vi "Measurement Logic.vi"() -> ()   [LabVIEW 2021, in "PSRR_PMIC.lvlib"]
uses:
  PSRR_PMIC.lvlib
  <vilib>/Plug-In SDKs/Measurements/Measure Call Context/Measure Call Context.lvclass
  Measurement Configuration.ctl
  Measurement Results.ctl
  <instrlib>/niDCPower/nidcpower.llb/niDCPower Output Function.ctl
  <instrlib>/niDCPower/nidcpower.llb/niDCPower Wait For Event - Event.ctl
  <instrlib>/niDCPower/nidcpower.llb/niDCPower Source Mode.ctl
  <instrlib>/niFgen/niFgen.llb/niFgen Output Mode.ctl
  <instrlib>/niScope/Controls/niScope vertical coupling.ctl
  <instrlib>/niScope/Controls/niScope trigger slope.ctl
  <instrlib>/niScope/Controls/niScope trigger coupling.ctl
  <instrlib>/niScope/Controls/niScope trigger source.ctl
  <instrlib>/niDCPower/nidcpower.llb/niDCPower Get Channel Name From String.vi
  <instrlib>/niScope/Utility/niScope Get Channel Name From String.vi
  <instrlib>/niScope/Configure/Trigger/niScope Configure Trigger Edge.vi
panel:
  out "measurement results":T1
  in  "measurement configuration":T2={"DUT setup time"=1.0, "Source resource name"="", "Source sense"=1009, "Source current limit"=0.15, "Source voltage level"=10.0, "Load resource name"="", "Load sense"=1009, "Load voltage limit range"=6.0, "Load current level"=0.025, "Fgen resource name"="", "Fgen channel name"="", "Fgen pk-pk amplitude"=1.0, "Fgen load impedance"=10000.0, "Fgen start frequency"=10.0, "Fgen stop frequency"=10000000.0, "Fgen frequency sweep points/points per decade"=10, "Fgen sweep type"="Logarithmic", "Fgen standard Waveform"=enum."Sine", "Scope resource name"="", "Scope input channel name"="", "Scope output channel name"="", "Scope probe attenuation"=1.0, "Scope samples per cycle"=1000, "Scope cycles to average"=4} {"Fgen stop frequency" format="%#_6p"; "Fgen pk-pk amplitude" format="%#_6p"; "Load sense" items=["Local"=1008, "Remote"=1009]; "Source sense" items=["Local"=1008, "Remote"=1009]}
  out "measure call context out":refnum<class "Measure Call Context.lvclass">
  in  "measure call context in":refnum<class "Measure Call Context.lvclass">
  out "error out":errorcluster
  in  "error in":errorcluster
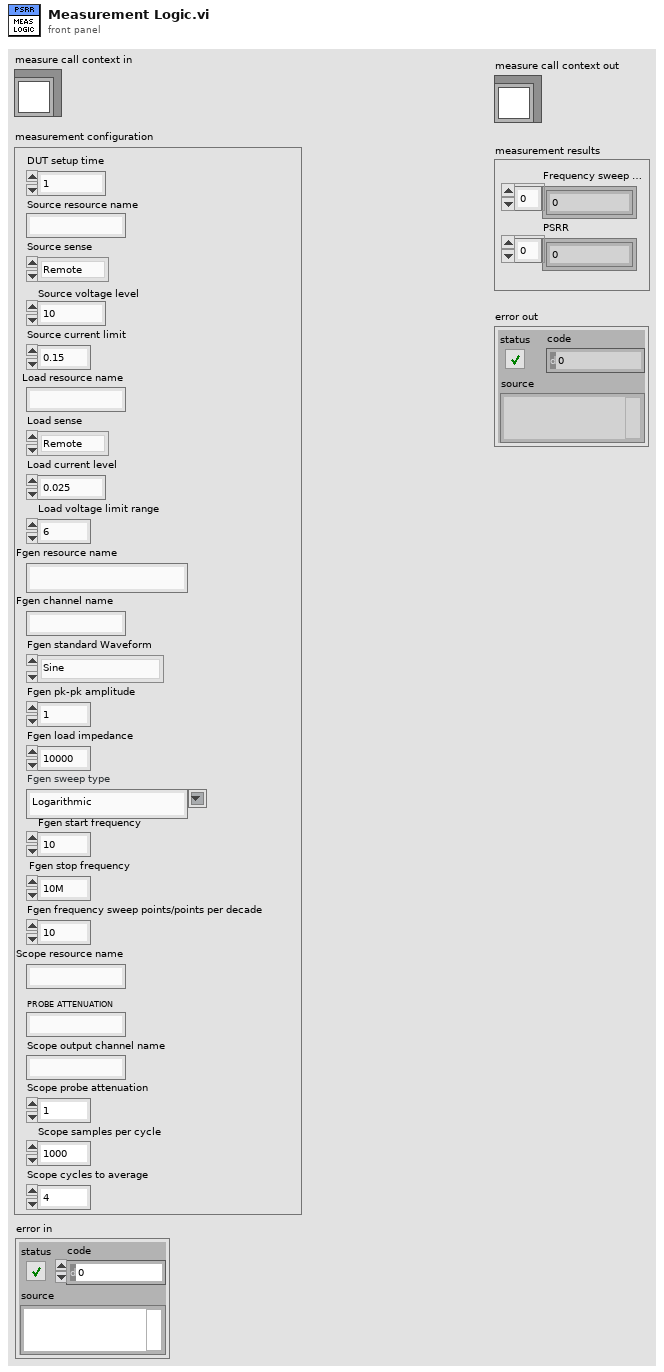
[diagram p1: front panel]
types:
  T1 = typedef "PSRR_PMIC.lvlib/Measurement Results.ctl" = cluster{"Frequency sweep points":dbl[], "PSRR":dbl[]}
  T2 = typedef "PSRR_PMIC.lvlib/Measurement Configuration.ctl" = cluster{"DUT setup time":dbl, "Source resource name":string, "Source sense":i32, "Source current limit":dbl, "Source voltage level":dbl, "Load resource name":string, "Load sense":i32, "Load voltage limit range":dbl, "Load current level":dbl, "Fgen resource name":string, "Fgen channel name":string, "Fgen pk-pk amplitude":dbl, "Fgen load impedance":dbl, "Fgen start frequency":dbl, "Fgen stop frequency":dbl, "Fgen frequency sweep points/points per decade":i32, "Fgen sweep type":string, "Fgen standard Waveform":enum32{"Sine", "Square", "Triangle", "Ramp Up", "Ramp Down", "DC", "Noise"}, "Scope resource name":string, "Scope input channel name":string, "Scope output channel name":string, "Scope probe attenuation":dbl, "Scope samples per cycle":i32, "Scope cycles to average":i32}
  T3 = typedef "niScope trigger coupling.ctl" = u16
  T4 = typedef "niScope trigger slope.ctl" = i32
  T5 = typedef "niScope vertical coupling.ctl" = i32
  T6 = typedef "niFgen Output Mode.ctl" = u32
  T7 = typedef "niDCPower Output Function.ctl" = i32
  T8 = typedef "niDCPower Source Mode.ctl" = i32
  T9 = typedef "niDCPower Wait For Event - Event.ctl" = i32
  T10 = enum32{"Sine", "Square", "Triangle", "Ramp Up", "Ramp Down", "DC", "Noise"}
  T11 = typedef "niScope trigger source.ctl" = string
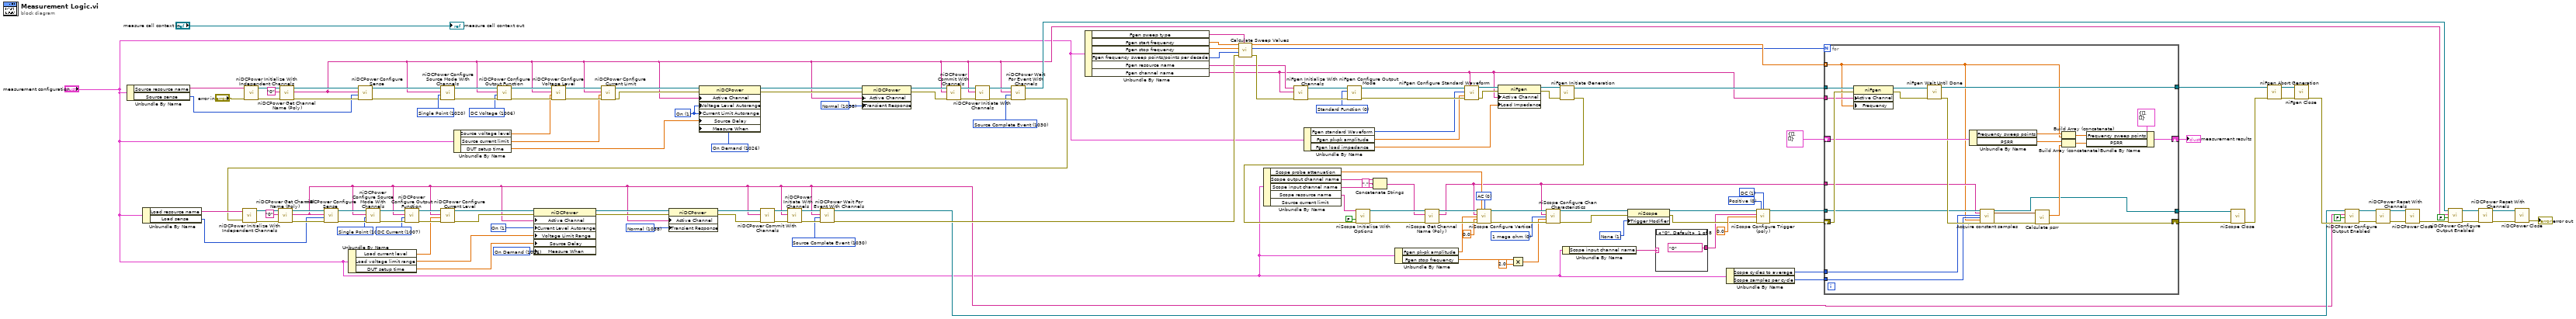
[diagram p0: block diagram]
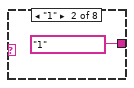
[diagram p2: hidden frame]
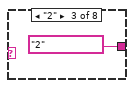
[diagram p3: hidden frame]
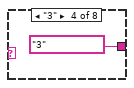
[diagram p4: hidden frame]
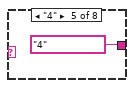
[diagram p5: hidden frame]
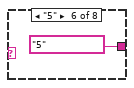
[diagram p6: hidden frame]
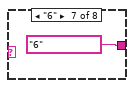
[diagram p7: hidden frame]
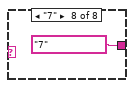
[diagram p8: hidden frame]
diagram:
  w53 = 1 items=["None"=1, "Auto Trigger"=2] ("Triggering:Trigger Modifier")
  w59 = T3 1 items=["AC"=0, "DC"=1, "HF Reject"=3, "LF Reject"=4, "AC Plus HF Reject"=1001] ("trigger coupling")
  w60 = T4 0 items=["Positive", "Negative"] ("trigger slope")
  w62 = T5 0 items=["AC", "DC", "Ground"] ("vertical coupling")
  w65 = u32 0 items=["1 mega ohm"=0, "50 ohms"=2] ("input impedance")
  w81 = T6 0 items=["Standard Function", "Frequency List", "Arbitrary Waveform", "Arbitrary Sequence", "Script"] ("Output Mode (default: 0=Standard Function)")
  w100 = T7 1007 items=["DC Voltage"=1006, "DC Current"=1007, "Pulse Voltage"=1049, "Pulse Current"=1050] ("output function")
  w101 = T8 1020 items=["Single Point"=1020, "Sequence"=1021] ("source mode")
  w26 = 1026 items=["Automatically after Source Complete"=1025, "On Demand"=1026, "On Measure Trigger"=1027] ("Measurement:Advanced:Measure When")
  w103 = 1 items=["Off", "On"] ("Source:DC Current:Current Level Autorange")
  w115 = 1038 items=["Slow"=1041, "Normal"=1038, "Fast"=1039, "Custom"=1042] ("Source:Transient Response")
  w118 = T9 1030 items=["Source Complete Event"=1030, "Measure Complete Event"=1031, "Sequence Iteration Complete Event"=1032, "Sequence Engine Done Event"=1033, "Pulse Complete Event"=1051, "Ready For Pulse Trigger Event"=1052] ("event")
  w123 = T9 1030 items=["Source Complete Event"=1030, "Measure Complete Event"=1031, "Sequence Iteration Complete Event"=1032, "Sequence Engine Done Event"=1033, "Pulse Complete Event"=1051, "Ready For Pulse Trigger Event"=1052] ("event")
  w131 = 1038 items=["Slow"=1041, "Normal"=1038, "Fast"=1039, "Custom"=1042] ("Source:Transient Response")
  w138 = 1026 items=["Automatically after Source Complete"=1025, "On Demand"=1026, "On Measure Trigger"=1027] ("Measurement:Advanced:Measure When")
  w144 = 1 items=["Off", "On"] ("Source:DC Voltage:Current Limit Autorange")
  w146 = T7 1006 items=["DC Voltage"=1006, "DC Current"=1007, "Pulse Voltage"=1049, "Pulse Current"=1050] ("output function")
  w149 = T8 1020 items=["Single Point"=1020, "Sequence"=1021] ("source mode")
  n1 = Unbundle By Name("measurement configuration") -> ("Source resource name"=w150:string, "Source sense"=w1:i32)
  n2 = Unbundle By Name("measurement configuration") -> ("Load resource name"=w91:string, "Load sense"=w2:i32)
  n3 = call <instrlib>:"niDCPower Initialize With Independent Channels.vi"("error in (no error)"="error in", "resource name"=w150) -> ("error out"=w152:errorcluster, "instrument handle out"=w153:refnum<k15>)  [unwired: 8 in]
  n4 = call-poly <instrlib>:"niDCPower Get Channel Name (Poly).vi"("error in (no error)"=w152, "index"="0", "instrument handle"=w153) -> ("error out"=w121:errorcluster, "name"=w10:string, "instrument handle out"=w122:refnum<k15>)  [unwired: 6 in]
  n5 = Unbundle By Name("measurement configuration") -> ("Load current level"=w102:dbl, "Load voltage limit range"=w97:dbl, "DUT setup time"=w112:dbl)
  n6 = call <instrlib>:"niDCPower Configure Sense.vi"("error in (no error)"=w121, "sense"=w1, "channel name"=w10, "instrument handle"=w122) -> ("error out"=w130:errorcluster, "instrument handle out"=w129:refnum<k15>)  [unwired: 6 in]
  n7 = call <instrlib>:"niDCPower Configure Source Mode With Channels.vi"("error in (no error)"=w130, "source mode"=w149, "channel name"=w10, "instrument handle"=w129) -> ("error out"=w148:errorcluster, "instrument handle out"=w147:refnum<k15>)  [unwired: 6 in]
  n8 = Unbundle By Name("measurement configuration") -> ("Source voltage level"=w127:dbl, "Source current limit"=w128:dbl, "DUT setup time"=w126:dbl)
  n9 = call <instrlib>:"niDCPower Configure Output Function.vi"("error in (no error)"=w148, "output function"=w146, "channel name"=w10, "instrument handle"=w147) -> ("error out"=w142:errorcluster, "instrument handle out"=w141:refnum<k15>)  [unwired: 6 in]
  n10 = call <instrlib>:"niDCPower Configure Voltage Level.vi"("error in (no error)"=w142, "voltage level"=w127, "channel name"=w10, "instrument handle"=w141) -> ("error out"=w139:errorcluster, "instrument handle out"=w140:refnum<k15>)  [unwired: 6 in]
  n11 = call <instrlib>:"niDCPower Configure Current Limit.vi"("error in (no error)"=w139, "current limit"=w128, "channel name"=w10, "instrument handle"=w140) -> ("error out"=w145:errorcluster, "instrument handle out"=w143:refnum<k15>)  [unwired: 6 in]
  n12 = property class="niDCPower"(reference=w143, error in=w145, "Active Channel"=w10, "Voltage Level Autorange"=w144, "Current Limit Autorange"=w144, "Source Delay"=w126, "Measure When"=w138) -> (reference out=w135:refnum<k15>, error out=w134:errorcluster)
  n13 = property class="niDCPower"(reference=w135, error in=w134, "Active Channel"=w10, "Transient Response"=w131) -> (reference out=w133:refnum<k15>, error out=w132:errorcluster)
  n14 = call <instrlib>:"niDCPower Commit With Channels.vi"("error in (no error)"=w132, "channel name"=w10, "instrument handle"=w133) -> ("error out"=w136:errorcluster, "instrument handle out"=w137:refnum<k15>)  [unwired: 7 in]
  n15 = call <instrlib>:"niDCPower Initiate With Channels.vi"("error in (no error)"=w136, "channel name"=w10, "instrument handle"=w137) -> ("error out"=w124:errorcluster, "instrument handle out"=w125:refnum<k15>)  [unwired: 7 in]
  n16 = call <instrlib>:"niDCPower Wait For Event With Channels.vi"("error in (no error)"=w124, "event"=w123, "channel name"=w10, "instrument handle"=w125) -> ("error out"=w72:errorcluster, "instrument handle out"=w13:refnum<k15>)  [unwired: 6 in]
  n17 = call <instrlib>:"niDCPower Initialize With Independent Channels.vi"("error in (no error)"=w72, "resource name"=w91) -> ("error out"=w95:errorcluster, "instrument handle out"=w96:refnum<k15>)  [unwired: 8 in]
  n18 = call-poly <instrlib>:"niDCPower Get Channel Name (Poly).vi"("error in (no error)"=w95, "index"="0", "instrument handle"=w96) -> ("error out"=w92:errorcluster, "name"=w11:string, "instrument handle out"=w93:refnum<k15>)  [unwired: 6 in]
  n19 = call <instrlib>:"niDCPower Configure Sense.vi"("error in (no error)"=w92, "sense"=w2, "channel name"=w11, "instrument handle"=w93) -> ("error out"=w106:errorcluster, "instrument handle out"=w109:refnum<k15>)  [unwired: 6 in]
  n20 = call <instrlib>:"niDCPower Configure Source Mode With Channels.vi"("error in (no error)"=w106, "source mode"=w101, "channel name"=w11, "instrument handle"=w109) -> ("error out"=w105:errorcluster, "instrument handle out"=w108:refnum<k15>)  [unwired: 6 in]
  n21 = call <instrlib>:"niDCPower Configure Output Function.vi"("error in (no error)"=w105, "output function"=w100, "channel name"=w11, "instrument handle"=w108) -> ("error out"=w104:errorcluster, "instrument handle out"=w107:refnum<k15>)  [unwired: 6 in]
  n22 = call <instrlib>:"niDCPower Configure Current Level.vi"("error in (no error)"=w104, "current level"=w102, "channel name"=w11, "instrument handle"=w107) -> ("error out"=w98:errorcluster, "instrument handle out"=w99:refnum<k15>)  [unwired: 6 in]
  n23 = property class="niDCPower"(reference=w99, error in=w98, "Active Channel"=w11, "Current Level Autorange"=w103, "Voltage Limit Range"=w97, "Source Delay"=w112, "Measure When"=w26) -> (reference out=w114:refnum<k15>, error out=w113:errorcluster)
  n24 = property class="niDCPower"(reference=w114, error in=w113, "Active Channel"=w11, "Transient Response"=w115) -> (reference out=w111:refnum<k15>, error out=w110:errorcluster)
  n25 = call <instrlib>:"niDCPower Commit With Channels.vi"("error in (no error)"=w110, "channel name"=w11, "instrument handle"=w111) -> ("error out"=w116:errorcluster, "instrument handle out"=w117:refnum<k15>)  [unwired: 7 in]
  n26 = call <instrlib>:"niDCPower Initiate With Channels.vi"("error in (no error)"=w116, "channel name"=w11, "instrument handle"=w117) -> ("error out"=w120:errorcluster, "instrument handle out"=w119:refnum<k15>)  [unwired: 7 in]
  n27 = call <instrlib>:"niDCPower Wait For Event With Channels.vi"("error in (no error)"=w120, "event"=w118, "channel name"=w11, "instrument handle"=w119) -> ("error out"=w79:errorcluster, "instrument handle out"=w12:refnum<k15>)  [unwired: 6 in]
  n28 = Unbundle By Name("measurement configuration") -> ("Fgen sweep type"=w78:string, "Fgen start frequency"=w27:dbl, "Fgen stop frequency"=w77:dbl, "Fgen frequency sweep points/points per decade"=w76:i32, "Fgen resource name"=w8:string, "Fgen channel name"=w7:string)
  n29 = call "Calculate Sweep Values.vi"("Sweep type"=w78, "error in"=w79, "Points"=w76, "Stop level"=w77, "Start level"=w27) -> ("error out"=w80:errorcluster, "Sweep points"=w30:i32, "Sweep values"=w31:dbl[])  [unwired: 4 in]
  n30 = Unbundle By Name("measurement configuration") -> ("Scope probe attenuation"=w48:dbl, "Scope output channel name"=w45:string, "Scope input channel name"=w47:string, "Scope resource name"=w61:string)  [unwired: 1 out]
  n31 = call <instrlib>:"niFgen Initialize With Channels.vi"("error in (no error)"=w80, "Channel Name"=w7, "Resource Name"=w8) -> ("error out"=w86:errorcluster, "Instrument Handle Out"=w89:refnum<k15>)  [unwired: 7 in]
  n32 = Unbundle By Name("measurement configuration") -> ("Fgen standard Waveform"=w74:T10, "Fgen pk-pk amplitude"=w73:dbl, "Fgen load impedance"=w75:dbl)
  n33 = call <instrlib>:"niFgen Configure Output Mode.vi"("error in (no error)"=w86, "Output Mode (default: 0=Standard Function)"=w81, "Instrument Handle"=w89) -> ("error out"=w85:errorcluster, "Instrument Handle Out"=w88:refnum<k15>)  [unwired: 6 in]
  n34 = Concatenate Strings(w45, "," ("string"), w47) -> (w44:string)
  n35 = Unbundle By Name("measurement configuration") -> ("Fgen pk-pk amplitude"=w6:dbl, "Fgen stop frequency"=w51:dbl)
  n36 = call <instrlib>:"niFgen Configure Standard Waveform.vi"("Instrument Handle"=w88, "Channel Name"=w7, "Waveform"=w74, "Amplitude"=w73, "error in (no error)"=w85) -> ("Instrument Handle Out"=w87:refnum<k15>, "error out"=w84:errorcluster)  [unwired: 9 in]
  n37 = property class="niFgen"(reference=w87, error in=w84, "Active Channel"=w7, "Load Impedance"=w75) -> (reference out=w83:refnum<k15>, error out=w82:errorcluster)
  n38 = Multiply(x=w51, y=2.0) -> (x*y=w52:dbl)
  n39 = call <instrlib>:"niFgen Initiate Generation.vi"("error in (no error)"=w82, "Instrument Handle"=w83) -> ("error out"=w49:errorcluster, "Instrument Handle Out"=w32:refnum<k15>)  [unwired: 8 in]
  n40 = call <instrlib>:"niScope Initialize With Options.vi"("resource name"=w61, "reset device"=FALSE, "error in"=w49) -> ("instrument handle"=w71:refnum<k15>, "error out"=w68:errorcluster)  [unwired: 11 in]
  n41 = call-poly <instrlib>:"niScope Get Channel Name (Poly).vi"("instrument handle"=w71, "index"=w44, "error in"=w68) -> ("instrument handle out"=w70:refnum<k15>, "channel name"=w33:string, "error out"=w67:errorcluster)  [unwired: 10 in]
  n42 = call <instrlib>:"niScope Configure Vertical.vi"("instrument handle"=w70, "probe attenuation"=w48, "vertical coupling"=w62, "channels"=w33, "vertical range"=w6, "vertical offset"=0.0, "error in"=w67) -> ("instrument handle out"=w69:refnum<k15>, "error out"=w66:errorcluster)  [unwired: 7 in]
  n43 = call <instrlib>:"niScope Configure Chan Characteristics.vi"("instrument handle"=w69, "channels"=w33, "input impedance"=w65, "maximum input frequency"=w52, "error in"=w66) -> ("instrument handle out"=w57:refnum<k15>, "error out"=w56:errorcluster)  [unwired: 9 in]
  n44 = Unbundle By Name("measurement configuration") -> ("Scope input channel name"=w3:string)
  n45 = property on="Property Node" class="niScope"(reference=w57, error in=w56, "Trigger Modifier"=w53) -> (reference out=w55:refnum<k15>, error out=w54:errorcluster)
  n46 = case shown="\"0\", Default" w3 {
    tunnel: [T11 "0" ("trigger source") T11 "1" ("trigger source") T11 "2" ("trigger source") T11 "3" ("trigger source") T11 "4" ("trigger source") T11 "5" ("trigger source") T11 "6" ("trigger source") T11 "7" ("trigger source")] -> w4
    frame "0", Default {
    }
    frame "1" {
    }
    frame "2" {
    }
    frame "3" {
    }
    frame "4" {
    }
    frame "5" {
    }
    frame "6" {
    }
    frame "7" {
    }
  }
  n47 = Unbundle By Name("measurement configuration") -> ("Scope cycles to average"=w43:i32, "Scope samples per cycle"=w42:i32)
  n48 = call-poly <instrlib>:"niScope Configure Trigger (poly).vi"("instrument handle"=w55, "trigger slope"=w60, "trigger coupling"=w59, "trigger source"=w4, "trigger level"=0.0, "error in"=w54) -> ("instrument handle out"=w34:refnum<k15>, "error out"=w35:errorcluster)  [unwired: 8 in]
  n49 = for {
    N: w30 -> [_]
    tunnel: w32 -> [w184]
    tunnel: w43 -> [w165]
    tunnel: w42 -> [w164]
    tunnel: w33 -> [w166]
    tunnel: w31 -> [w163] mode=indexing
    shift-right: [w172] -> w37
    shift-left: w35 -> [w183]
    tunnel: [w182] -> w38
    tunnel: [w168] -> w36
    tunnel: w34 -> [w167]
    shift-right: [w180] -> w29
    shift-left: T1 {"Frequency sweep points"=[], "PSRR"=[]} ("Measurement Results") -> [w179]
    tunnel: w7 -> [w174]
    n50 = property class="niFgen"(reference=w184, error in=w183, "Active Channel"=w174, "Frequency"=w163) -> (reference out=w185:refnum<k15>, error out=w186:errorcluster)
    n51 = call <instrlib>:"niFgen Wait Until Done.vi"("error in (no error)"=w186, "Instrument Handle"=w185) -> ("error out"=w171:errorcluster, "Instrument Handle Out"=w182:refnum<k15>)  [unwired: 8 in]
    n52 = Unbundle By Name(w179) -> ("Frequency sweep points"=w178:dbl[], "PSRR"=w177:dbl[])
    n53 = call "Acquire constant samples.vi"("Instrument handle"=w167, "Channel(s)"=w166, "Cycles to acquire"=w165, "Samples/cycle"=w164, "Frequency"=w163, "error in (no error)"=w171) -> ("Instrument handle out"=w168:refnum<k15>, "Waveform(s)"=w169:waveform(dbl)[], "error out"=w170:errorcluster)  [unwired: 11 in]
    n54 = call "Calculate psrr.vi"("error in (no error)"=w170, "Time signal(s) in"=w169) -> ("error out"=w172:errorcluster, "PSRR"=w173:dbl)  [unwired: 8 in]
    n55 = Build Array (concatenate)(w178, w163) -> (w176:dbl[])
    n56 = Build Array (concatenate)(w177, w173) -> (w175:dbl[])
    n57 = Bundle By Name(cluster=T1 {"Frequency sweep points"=[], "PSRR"=[]} ("Measurement Results"), "Frequency sweep points"=w176, "PSRR"=w175) -> (w180:T1)
  }
  "measurement results" <- w29
  n58 = call <instrlib>:"niScope Close.vi"("instrument handle"=w36, "error in"=w37) -> ("error out"=w41:errorcluster)  [unwired: 13 in]
  n59 = call <instrlib>:"niFgen Abort Generation.vi"("error in (no error)"=w41, "Instrument Handle"=w38) -> ("error out"=w40:errorcluster, "Instrument Handle Out"=w39:refnum<k15>)  [unwired: 8 in]
  n60 = call <instrlib>:"niFgen Close.vi"("error in (no error)"=w40, "Instrument Handle"=w39) -> ("error out"=w14:errorcluster)  [unwired: 9 in]
  n61 = call <instrlib>:"niDCPower Configure Output Enabled.vi"("error in (no error)"=w14, "output enabled"=FALSE, "channel name"=w11, "instrument handle"=w12) -> ("error out"=w19:errorcluster, "instrument handle out"=w18:refnum<k15>)  [unwired: 6 in]
  n62 = call <instrlib>:"niDCPower Reset With Channels.vi"("error in (no error)"=w19, "instrument handle"=w18) -> ("error out"=w16:errorcluster, "instrument handle out"=w17:refnum<k15>)  [unwired: 8 in]
  n63 = call <instrlib>:"niDCPower Close.vi"("error in (no error)"=w16, "instrument handle"=w17) -> ("error out"=w20:errorcluster)  [unwired: 9 in]
  n64 = call <instrlib>:"niDCPower Configure Output Enabled.vi"("error in (no error)"=w20, "output enabled"=FALSE, "channel name"=w10, "instrument handle"=w13) -> ("error out"=w21:errorcluster, "instrument handle out"=w22:refnum<k15>)  [unwired: 6 in]
  n65 = call <instrlib>:"niDCPower Reset With Channels.vi"("error in (no error)"=w21, "instrument handle"=w22) -> ("error out"=w24:errorcluster, "instrument handle out"=w25:refnum<k15>)  [unwired: 8 in]
  n66 = call <instrlib>:"niDCPower Close.vi"("error in (no error)"=w24, "instrument handle"=w25) -> ("error out"=→"error out":errorcluster)  [unwired: 9 in]
  "measure call context out" <- "measure call context in"
